vi "Test TX to Multi RX.vi"() -> ()   [LabVIEW 2021]
uses:
  <vilib>/CIF Foundation/CIF CAN RW Core/typedef/CAN Port Configuration.ctl
  <vilib>/CIF Foundation/CIF CAN RW Core/typedef/CAN Mode.ctl
  <vilib>/CIF Foundation/CIF CAN RW Core/typedef/FD Config.ctl
  <vilib>/xnet/xnet.llb/XNET Frame CAN.ctl
  <vilib>/xnet/xnet.llb/XNET Frame Type CAN.ctl
  typedef/Time Pair.ctl
  <vilib>/CIF Foundation/CIF CAN RW Core/typedef/Statistics.ctl
  XNET CAN RW.lvclass
  C:/Program Files/National Instruments/LabVIEW 2021/vi.lib/CIF Foundation/CIF CAN RW Core/CAN_RW_CORE.lvclass
  XNET CAN RW.lvclass/XNET CAN RW.ctl
  <vilib>/CIF Foundation/CIF CAN RW Core/CAN_RW_CORE.lvclass/CAN_RW_CORE.ctl
  <vilib>/CIF Foundation/CIF Utilities/Time/System Time/LabVIEW Time to TAI Time.vi
  Utilities/Add Error.vi
  <vilib>/CIF Foundation/CIF Utilities/Time/System Time/Get System Time.vi
  <vilib>/xnet/xnet.llb/XNET Read.vi
  <vilib>/xnet/xnet.llb/XNET Read (State Time Start).vi
  Utilities/Add Error Core.vi
  <vilib>/xnet/xnet.llb/XNET Read (State Time Current).vi
  <vilib>/CIF Foundation/CIF CAN RW Core/CAN_RW_CORE.lvclass
panel:
  out "Plugin Status":string[][](table)
  out "Statistcs":T1
  out "Time Delta":i64
  out "Time Pair":T2
  out "Local CAN":T3[](array[typedef]) {"payload" format="%x"; "timestamp" format="%<%.7X\n%x>T"; "type" items=["CAN Data"=0, "CAN Remote"=1, "CAN Bus Error"=2, "CAN 2.0 Data"=8, "CAN FD Data"=16, "CAN FD+BRS Data"=24, "J1939 Data"=192, "Delay"=224, "Log Trigger"=225, "Start Trigger"=226]; "identifier" format="%x"}
  out "Local Subordinate":T3[](array[typedef]) {"payload" format="%x"; "timestamp" format="%<%.7X\n%x>T"; "type" items=["CAN Data"=0, "CAN Remote"=1, "CAN Bus Error"=2, "CAN 2.0 Data"=8, "CAN FD Data"=16, "CAN FD+BRS Data"=24, "J1939 Data"=192, "Delay"=224, "Log Trigger"=225, "Start Trigger"=226]; "identifier" format="%x"}
  out "Remote CAN":T3[](array[typedef]) {"payload" format="%x"; "timestamp" format="%<%.7X\n%x>T"; "type" items=["CAN Data"=0, "CAN Remote"=1, "CAN Bus Error"=2, "CAN 2.0 Data"=8, "CAN FD Data"=16, "CAN FD+BRS Data"=24, "J1939 Data"=192, "Delay"=224, "Log Trigger"=225, "Start Trigger"=226]; "identifier" format="%x"}
  in  "XNET CAN Data":T3[](array[typedef])=[{"timestamp"=timestamp(3831573600 s since 1904-01-01), "payload"=[1, 2, 3, 4, 5, 6, 7, 8], "identifier"=33, "type"=16, "extended?"=TRUE, "echo?"=FALSE}, {"timestamp"=timestamp(3831570000 s since 1904-01-01), "payload"=[10, 11, 10, 13, 11, 10, 11, 14], "identifier"=82, "type"=0, "extended?"=TRUE, "echo?"=FALSE}] {"payload" format="%x"; "timestamp" format="%<%.7X\n%x>T"; "type" items=["CAN Data"=0, "CAN Remote"=1, "CAN Bus Error"=2, "CAN 2.0 Data"=8, "CAN FD Data"=16, "CAN FD+BRS Data"=24, "J1939 Data"=192, "Delay"=224, "Log Trigger"=225, "Start Trigger"=226]; "identifier" format="%x"}
  out "Pass":bool
  out "error out":errorcluster
  in  "Port Configuration":T5={"Mode"=enum."CAN FD", "Baud Rate"=500000, "Temination On"=TRUE, "Subordinate"=FALSE, "Echo TX"=FALSE, "FD Config"={"FD Baud Rate"=2000000, "ISO Mode"=TRUE, "BRS Enabled"=TRUE}} {"FD Config"."FD Baud Rate" format="%.0p"; "Baud Rate" format="%.0p"}
  in  "RX Initerface":string="CAN2"
  in  "TX Interface":string="CAN1"
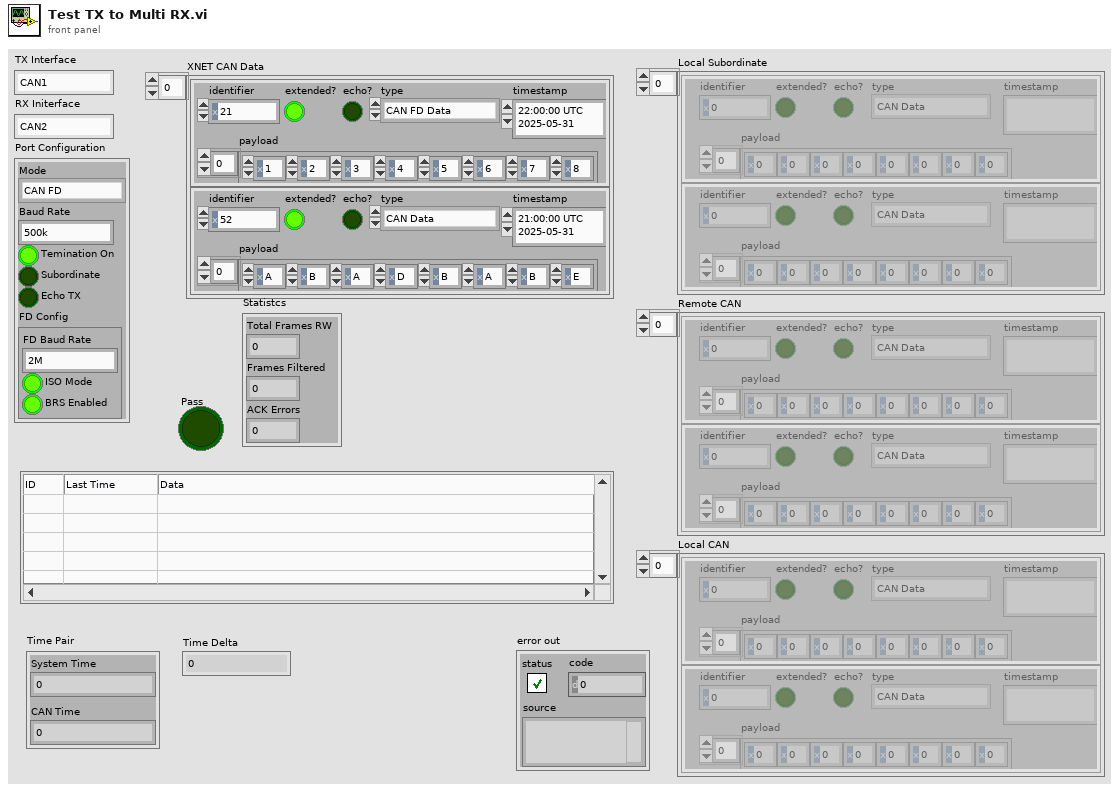
[diagram p1: front panel]
types:
  T1 = typedef "CAN_RW_CORE.lvclass/Statistics.ctl" = cluster{"Total Frames RW":u32, "Frames Filtered ":u32, "ACK Errors":u32}
  T2 = typedef "XNET CAN RW.lvclass/Time Pair.ctl" = cluster{"System Time":i64, "CAN Time":i64}
  T3 = typedef "XNET Frame CAN.ctl" = cluster{"timestamp":timestamp, "payload":u8[], "identifier":u32, "type":T4, "extended?":bool, "echo?":bool}
  T4 = typedef "XNET Frame Type CAN.ctl" = u8
  T5 = typedef "CAN_RW_CORE.lvclass/CAN Port Configuration.ctl" = cluster{"Mode":T6, "Baud Rate":u64, "Temination On":bool, "Subordinate":bool, "Echo TX":bool, "FD Config":T7}
  T6 = typedef "CAN_RW_CORE.lvclass/CAN Mode.ctl" = enum16{"CAN 2.0", "CAN FD"}
  T7 = typedef "CAN_RW_CORE.lvclass/FD Config.ctl" = cluster{"FD Baud Rate":u64, "ISO Mode":bool, "BRS Enabled":bool}
  T8 = typedef "XNET CAN RW.lvclass/CAN Return Map.ctl" = map{u32, T3}
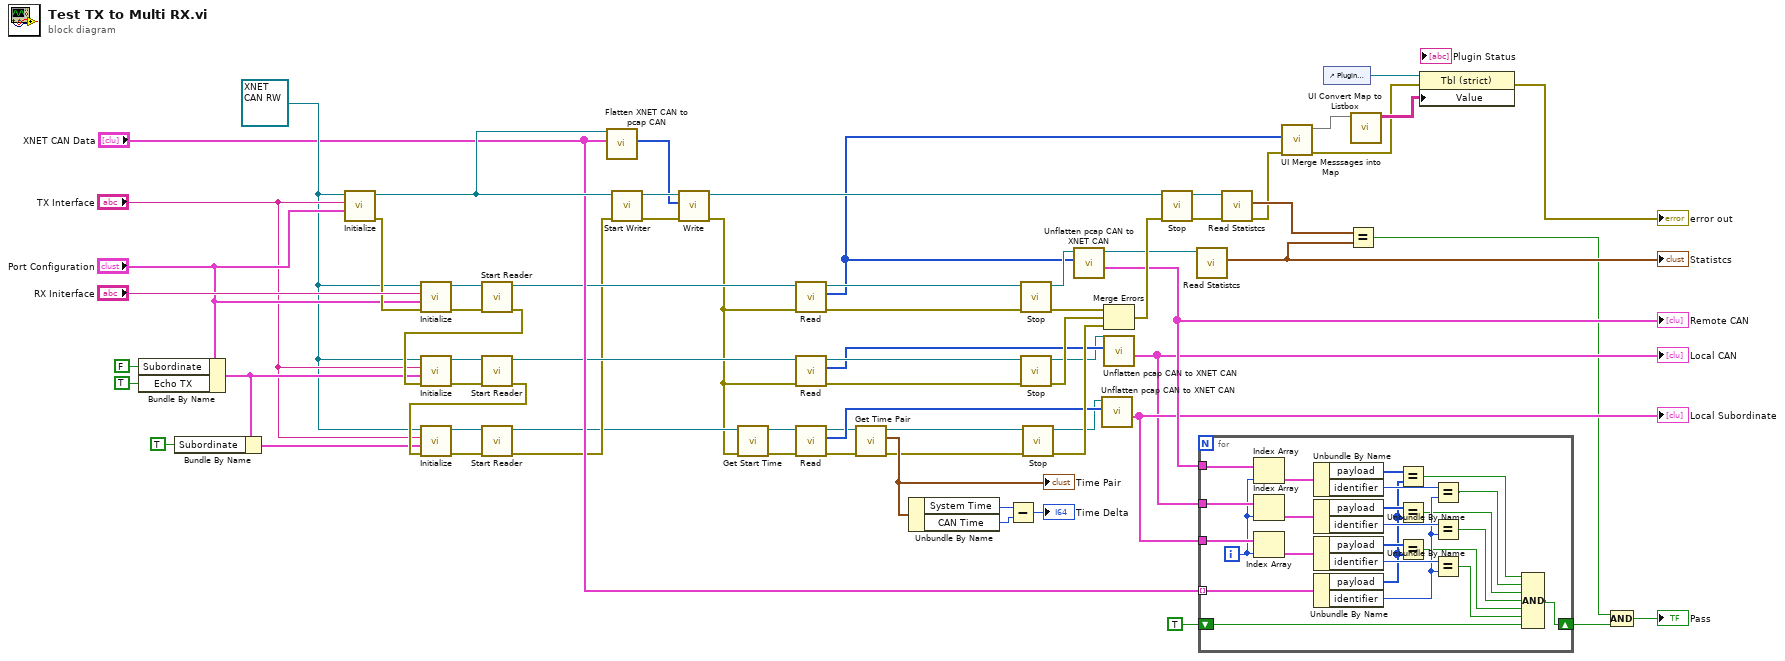
[diagram p0: block diagram]
diagram:
  w42 = refnum<class "XNET CAN RW.lvclass"> refnum ("CAN_Logic in")
  n1 = Bundle By Name(cluster="Port Configuration", "Subordinate"=FALSE, "Echo TX"=TRUE) -> (w50:T5)
  n2 = Bundle By Name(cluster=w50, "Subordinate"=TRUE) -> (w49:T5)
  n3 = call "Initialize.vi"("Port Configuration"="Port Configuration", "Interface"="TX Interface", "XNET_CAN_RW in"=w42) -> ("error out"=w70:errorcluster, "XNET_CAN_RW out"=w41:refnum<class "XNET CAN RW.lvclass">)  [unwired: 7 in]
  n4 = call "Initialize.vi"("error in (no error)"=w70, "Port Configuration"="Port Configuration", "Interface"="RX Initerface", "XNET_CAN_RW in"=w42) -> ("error out"=w68:errorcluster, "XNET_CAN_RW out"=w69:refnum<class "XNET CAN RW.lvclass">)  [unwired: 6 in]
  n5 = call-dynamic "Start Reader.vi"("error in (no error)"=w68, "XNET_CAN_RW in"=w69) -> ("error out"=w58:errorcluster, "XNET_CAN_RW out"=w22:refnum<class "XNET CAN RW.lvclass">)  [unwired: 8 in]
  n6 = call "Initialize.vi"("error in (no error)"=w58, "Port Configuration"=w50, "Interface"="TX Interface", "XNET_CAN_RW in"=w42) -> ("error out"=w60:errorcluster, "XNET_CAN_RW out"=w59:refnum<class "XNET CAN RW.lvclass">)  [unwired: 6 in]
  n7 = call-dynamic "Start Reader.vi"("error in (no error)"=w60, "XNET_CAN_RW in"=w59) -> ("error out"=w52:errorcluster, "XNET_CAN_RW out"=w21:refnum<class "XNET CAN RW.lvclass">)  [unwired: 8 in]
  n8 = call "Initialize.vi"("error in (no error)"=w52, "Port Configuration"=w49, "Interface"="TX Interface", "XNET_CAN_RW in"=w42) -> ("error out"=w53:errorcluster, "XNET_CAN_RW out"=w54:refnum<class "XNET CAN RW.lvclass">)  [unwired: 6 in]
  n9 = call-dynamic "Start Reader.vi"("error in (no error)"=w53, "XNET_CAN_RW in"=w54) -> ("error out"=w17:errorcluster, "XNET_CAN_RW out"=w16:refnum<class "XNET CAN RW.lvclass">)  [unwired: 8 in]
  n10 = call "Flatten XNET CAN to pcap CAN.vi"("XNET CAN Data"="XNET CAN Data", "XNET_CAN_RW in"=w41) -> ("pcap CAN DATA"=w31:u8[])  [unwired: 7 in, 2 out]
  n11 = call-dynamic "Start Writer.vi"("error in (no error)"=w17, "XNET_CAN_RW in"=w41) -> ("error out"=w66:errorcluster, "XNET_CAN_RW out"=w67:refnum<class "XNET CAN RW.lvclass">)  [unwired: 8 in]
  n12 = call-dynamic "Write.vi"("error in (no error)"=w66, "pcap CAN DATA in"=w31, "XNET_CAN_RW in"=w67) -> ("error out"=w15:errorcluster, "XNET_CAN_RW out"=w63:refnum<class "XNET CAN RW.lvclass">)  [unwired: 6 in, 1 out]
  n13 = call "Get Start Time.vi"("error in (no error)"=w15, "XNET CAN RW in"=w16) -> ("error out"=w14:errorcluster, "XNET CAN RW out"=w13:refnum<class "XNET CAN RW.lvclass">)  [unwired: 8 in]
  n14 = call-dynamic "Read.vi"("error in (no error)"=w15, "XNET_CAN_RW in"=w22) -> ("error out"=w64:errorcluster, "pcap CAN Data"=w4:u8[], "XNET_CAN_RW out"=w65:refnum<class "XNET CAN RW.lvclass">)  [unwired: 5 in, 2 out]
  n15 = call-dynamic "Read.vi"("error in (no error)"=w15, "XNET_CAN_RW in"=w21) -> ("error out"=w62:errorcluster, "pcap CAN Data"=w38:u8[], "XNET_CAN_RW out"=w61:refnum<class "XNET CAN RW.lvclass">)  [unwired: 5 in, 2 out]
  n16 = call-dynamic "Read.vi"("error in (no error)"=w14, "XNET_CAN_RW in"=w13) -> ("error out"=w26:errorcluster, "pcap CAN Data"=w36:u8[], "XNET_CAN_RW out"=w25:refnum<class "XNET CAN RW.lvclass">)  [unwired: 5 in, 2 out]
  n17 = call "Get Time Pair.vi"("error in (no error)"=w26, "XNET CAN RW in"=w25) -> ("error out"=w23:errorcluster, "Time Pair"=w30:T2, "XNET CAN RW out"=w24:refnum<class "XNET CAN RW.lvclass">)  [unwired: 7 in]
  "Time Pair" <- w30
  n18 = Unbundle By Name(w30) -> ("System Time"=w29:i64, "CAN Time"=w28:i64)
  n19 = Subtract(x=w29, y=w28) -> (x-y=→"Time Delta":i64)
  n20 = call-dynamic "Stop.vi"("error in (no error)"=w64, "XNET_CAN_RW in"=w65) -> ("error out"=w47:errorcluster, "XNET_CAN_RW out"=w40:refnum<class "XNET CAN RW.lvclass">)  [unwired: 8 in]
  n21 = call-dynamic "Stop.vi"("error in (no error)"=w62, "XNET_CAN_RW in"=w61) -> ("error out"=w46:errorcluster, "XNET_CAN_RW out"=w37:refnum<class "XNET CAN RW.lvclass">)  [unwired: 8 in]
  n22 = call-dynamic "Stop.vi"("error in (no error)"=w23, "XNET_CAN_RW in"=w24) -> ("error out"=w45:errorcluster, "XNET_CAN_RW out"=w35:refnum<class "XNET CAN RW.lvclass">)  [unwired: 8 in]
  n23 = call "Unflatten pcap CAN to XNET CAN.vi"("pcap CAN DATA in"=w4, "XNET_CAN_RW in"=w40) -> ("XNET CAN Data"=w39:T3[], "XNET_CAN_RW out"=w18:refnum<class "XNET CAN RW.lvclass">)  [unwired: 4 in, 4 out]
  "Remote CAN" <- w39
  n24 = call "Unflatten pcap CAN to XNET CAN.vi"("pcap CAN DATA in"=w36, "XNET_CAN_RW in"=w35) -> ("XNET CAN Data"=w34:T3[])  [unwired: 4 in, 5 out]
  "Local Subordinate" <- w34
  n25 = Merge Errors(w47, w46, w45) -> (w44:errorcluster)
  n26 = call "Unflatten pcap CAN to XNET CAN.vi"("pcap CAN DATA in"=w38, "XNET_CAN_RW in"=w37) -> ("XNET CAN Data"=w33:T3[])  [unwired: 4 in, 5 out]
  "Local CAN" <- w33
  n27 = call-dynamic "Stop.vi"("error in (no error)"=w44, "XNET_CAN_RW in"=w63) -> ("error out"=w19:errorcluster, "XNET_CAN_RW out"=w20:refnum<class "XNET CAN RW.lvclass">)  [unwired: 8 in]
  n28 = call <vilib>:"Read Statistcs.vi"("CAN_RW_CORE in"=w18) -> ("Statistcs"=w11:T1)  [unwired: 8 in, 2 out]
  "Statistcs" <- w11
  n29 = for {
    tunnel: "XNET CAN Data" -> [w95] mode=indexing
    tunnel: w34 -> [w76]
    tunnel: w33 -> [w75]
    tunnel: w39 -> [w78]
    shift-right: [w79] -> w10
    shift-left: TRUE -> [w80]
    i -> [w72]
    n30 = Index Array(array=w78, index=w72) -> (element=w77:T3)
    n31 = Index Array(array=w75, index=w72) -> (element=w74:T3)
    n32 = Index Array(array=w76, index=w72) -> (element=w73:T3)
    n33 = Unbundle By Name(w77) -> ("payload"=w94:u8[], "identifier"=w93:u32)
    n34 = Unbundle By Name(w74) -> ("payload"=w91:u8[], "identifier"=w92:u32)
    n35 = Unbundle By Name(w73) -> ("payload"=w90:u8[], "identifier"=w89:u32)
    n36 = Unbundle By Name(w95) -> ("payload"=w88:u8[], "identifier"=w87:u32)
    n37 = Equal?(x=w94, y=w88) -> (x = y?=w86:bool)
    n38 = Equal?(x=w91, y=w88) -> (x = y?=w84:bool)
    n39 = Equal?(x=w90, y=w88) -> (x = y?=w82:bool)
    n40 = Equal?(x=w93, y=w87) -> (x = y?=w85:bool)
    n41 = Equal?(x=w92, y=w87) -> (x = y?=w83:bool)
    n42 = Equal?(x=w89, y=w87) -> (x = y?=w81:bool)
    n43 = Compound Arithmetic op=AND(w86, w85, w84, w83, w82, w81, w80) -> (w79:bool)
  }
  n44 = call <vilib>:"Read Statistcs.vi"("error in (no error)"=w19, "CAN_RW_CORE in"=w20) -> ("error out"=w3:errorcluster, "Statistcs"=w12:T1)  [unwired: 7 in, 1 out]
  n45 = call "UI Merge Messsages into Map.vi"("error in (no error)"=w3, "pcap CAN DATA in"=w4) -> ("error out"=w5:errorcluster, "CAN Return MAP out"=w7:T8)  [unwired: 8 in]
  n46 = control-ref of="Plugin Status"() -> (w1:refnum<vi>)
  n47 = Equal?(x=w12, y=w11) -> (x = y?=w8:bool)
  n48 = call "UI Convert Map to Listbox.vi"("CAN Return MAP in"=w7) -> ("CAN Data for Mutli Listbox"=w6:string[][])  [unwired: 10 in]
  n49 = property class="Tbl (strict)"(reference=w1, error in=w5, "Value"=w6) -> (error out=→"error out":errorcluster)  [unwired: 1 out]
  n50 = Compound Arithmetic op=AND(w8, w10) -> (→"Pass":bool)
